vi "DVR Get StartDefault Languages.vi"(8 "error in (no error)":errorcluster) -> (0 "error out":errorcluster, 2 "Default":i32, 3 "Start":T1)   [LabVIEW 2019, in "Language Selection.lvlib"]
doc: "Converts the Data Value Reference back into Controls translation.\n- - -\nCopyright (c) 2026, Merecs Engineering GmbH"
uses:
  Language Selection.lvlib
  TypeDefs/Enum Language.ctl
  Global Language Selection.vi
panel:
  # "Connector Pane"
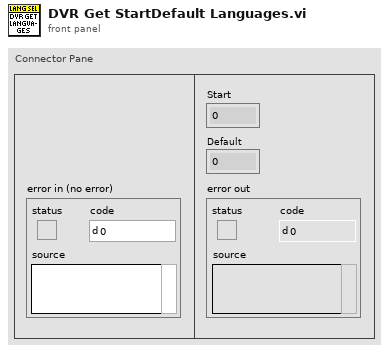
[diagram p1: front panel]
types:
  T1 = typedef "Language Selection.lvlib/Enum Language.ctl" = i32
  T2 = typedef "Language Selection.lvlib/Cluster DVR.ctl" = cluster{"Data":T3, "VIs":path[], "FP Translation":map{string, T4}, "Text Translation":map{string, T4}, "Front panels":set{refnum<vi>}}
  T3 = typedef "Language Selection.lvlib/Cluster Settings Data.ctl" = cluster{"Startup Language":string, "Default Language":string, "Languages":cluster{"ANSI":string[], "Unicode":string[]}}
  T4 = typedef "Language Selection.lvlib/Cluster LanguageClusterWithRefnum.ctl" = cluster{"Property":T5[], "Controls":set{refnum<vi>}}
  T5 = typedef "Language Selection.lvlib/Cluster PropertyTranslation.ctl" = cluster{"Type":T6, "Translation ANSI":string[], "Translation Unicode":string[]}
  T6 = typedef "Language Selection.lvlib/Enum Property Type.ctl" = enum16{"NA", "Caption", "String Value", "Boolean Text", "Ring Strings", "1D Array Elements", "2D Array Elements", "(MC)Listbox Header", "(MC)Listbox Items", "Tab Pages Names", "X & Y GraphChart", "Plot Names", "Table Headers", "Table Items", "TipStrip", "Combobox Strings", "Cursor Name", "Tree Col Headers"}
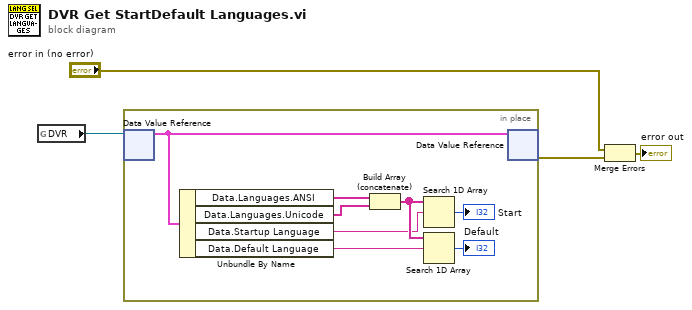
[diagram p0: block diagram]
diagram:
  n1 = global read "Global Language Selection.vi" "DVR"() -> (w1:refnum<data-value>)
  n2 = in-place "In Place Element Structure" {
    n3 = in-place-dvr #1(w1) -> (w12:T2)  [unwired: 1 out]
    n4 = Unbundle By Name(w12) -> ("Data.Languages.ANSI"=w11:string[], "Data.Languages.Unicode"=w10:string[], "Data.Startup Language"=w8:string, "Data.Default Language"=w7:string)
    n5 = Build Array (concatenate)(w11, w10) -> (w9:string[])
    n6 = Search 1D Array(1D array=w9, element=w8) -> (index of element=→"Start":i32)  [unwired: 1 in]
    n7 = Search 1D Array(1D array=w9, element=w7) -> (index of element=→"Default":i32)  [unwired: 1 in]
    n8 = in-place-dvr #1(w12) -> (w3:errorcluster)  [unwired: 1 out]
  }
  n9 = Merge Errors("error in (no error)", w3) -> (→"error out":errorcluster)
